vi "Panel.vi"(11 "ArrayHostPanel in":refnum<class "ArrayHostPanel.lvclass">) -> ()   [LabVIEW 2020, in "Nested.lvlib" / "ArrayHostPanel.lvclass"]
uses:
  ArrayHostPanel.lvclass
  OOPanel/Panel/Basic UI State.ctl
  OOPanel/Panel/Panel.lvclass
  OOPanel/OOPanel.lvlib
  OOPanel/ArrayManager/ArrayManager.lvclass
  ColorArrayPanel/ColorArrayPanel.lvclass
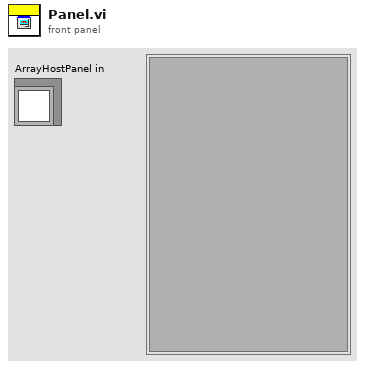
[diagram p1: front panel]
types:
  T1 = typedef "OOPanel.lvlib/Panel.lvclass/Basic UI State.ctl" = enum16{"Init", "Run", "Close"}
  T2 = typedef "OOPanel.lvlib/Panel.lvclass/Panel Events.ctl" = cluster{"Visbility":refnum<user-event>, "Close":refnum<user-event>}
  T3 = typedef "OOPanel.lvlib/Visibility State.ctl" = enum16{"Idle", "Closed", "Hidden", "Visible", "Subpanel", "Hidden Subpanel"}
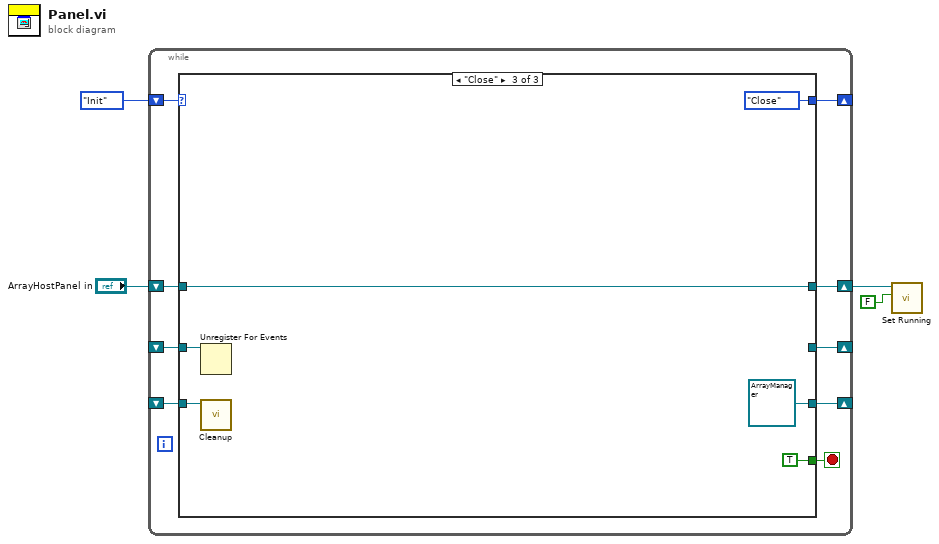
[diagram p0: block diagram]
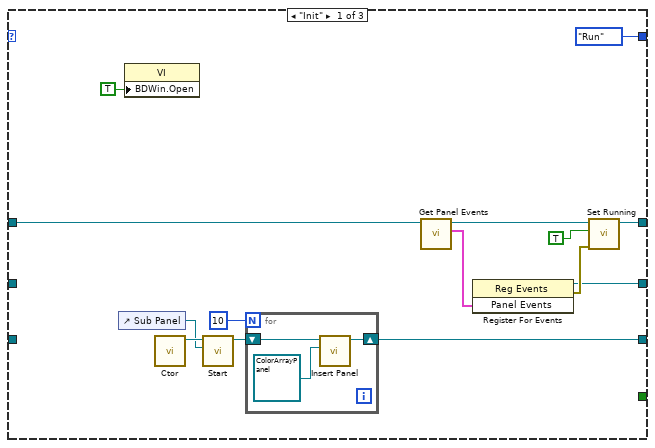
[diagram p2: hidden frame]
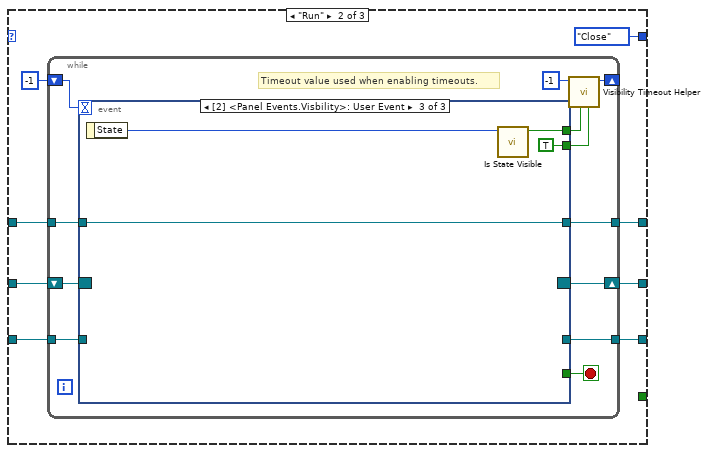
[diagram p3: hidden frame]
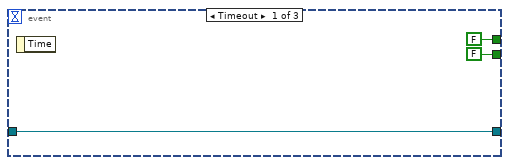
[diagram p4: hidden frame]
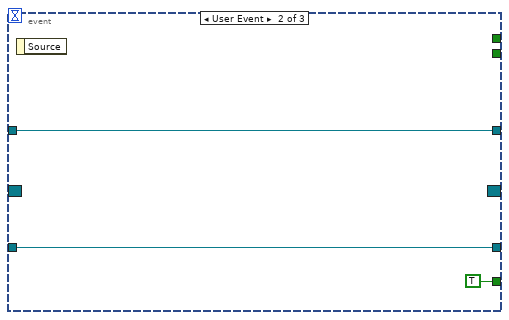
[diagram p5: hidden frame]
diagram:
  n1 = while {
    shift-right: [w12] -> _
    shift-left: _ -> [w13]
    shift-right: [w10] -> _
    shift-left: Basic_UI_State."Init" ("Basic UI State") -> [w11]
    shift-right: [w8] -> w1
    shift-left: "ArrayHostPanel in" -> [w7]
    shift-right: [w6] -> _
    shift-left: _ -> [w5]
    stop <- w9 stop-if-true
    n2 = case shown="\"Close\"" w11 {
      tunnel: w13 -> [_ w38 w64]
      tunnel: [w24 w36 _] -> w12
      tunnel: [Basic_UI_State."Run" ("Basic UI State") Basic_UI_State."Close" ("Basic UI State") Basic_UI_State."Close" ("Basic UI State")] -> w10
      tunnel: [_ _ TRUE] -> w9
      tunnel: [w23 w33 w61] -> w8
      tunnel: w7 -> [w22 w34 w61]
      tunnel: [w15 w31 refnum<class "ArrayManager.lvclass"> refnum ("ArrayManager out")] -> w6
      tunnel: w5 -> [_ w32 w63]
      frame "Init" {
        n3 = control-ref of="Sub Panel"() -> (w17:refnum<vi>)
        n4 = property class="VI"("BDWin.Open"=TRUE ("Block Diagram Window:Open")) -> ()  [unwired: 2 in, 2 out]
        n5 = call "Ctor.vi"() -> ("PanelArray"=w18:refnum<class "ArrayManager.lvclass">)  [unwired: 10 in, 1 out]
        n6 = call "Start.vi"("Container"=w17, "ArrayManager in"=w18) -> ("ArrayManager out"=w16:refnum<class "ArrayManager.lvclass">)  [unwired: 8 in, 1 out]
        n7 = for {
          N: 10 -> [_]
          shift-right: [w28] -> w15
          shift-left: w16 -> [w30]
          n8 = call "Insert Panel.vi"("Panel/Type"=refnum<class "ColorArrayPanel.lvclass"> refnum ("Nested.lvlib:ColorArrayPanel.lvclass"), "PanelArray in"=w30) -> ("PanelArray out"=w28:refnum<class "ArrayManager.lvclass">)  [unwired: 7 in, 2 out]
        }
        n9 = call "Get Panel Events.vi"("Panel in"=w22) -> ("Panel Events"=w20:T2, "Panel out"=w21:refnum<class "ArrayHostPanel.lvclass">)  [unwired: 8 in, 1 out]
        n10 = register-events(w20) -> (reference out=w24:refnum<event-registration>, error out=w26:errorcluster)  [unwired: 2 in]
        n11 = call "Set Running.vi"("error in (no error)"=w26, "Running"=TRUE, "Panel in"=w21) -> ("Panel out"=w23:refnum<class "ArrayHostPanel.lvclass">)  [unwired: 7 in, 1 out]
      }
      frame "Run" {
        n12 = while {
          shift-right: [w46] -> w36
          shift-left: w38 -> [w47]
          shift-right: [w49] -> _
          shift-left: -1 ("Timeout") -> [w48]
          tunnel: w34 -> [w42]
          tunnel: [w41] -> w33
          tunnel: w32 -> [w40]
          tunnel: [w39] -> w31
          stop <- w43 stop-if-true
          # "Timeout value used when enabling timeouts."
          n13 = event shown="[2] <Panel Events.Visbility>: User Event" {
            selector: w47 -> [_ _ _]
            dyn-events: [_ _ _] -> w46
            timeout: w48 -> [_ _ _]
            tunnel: [FALSE _ w59] -> w45
            tunnel: [FALSE _ TRUE] -> w44
            tunnel: [_ TRUE _] -> w43
            tunnel: w42 -> [w51 w55 w57]
            tunnel: [w51 w55 w57] -> w41
            tunnel: w40 -> [_ w54 _]
            tunnel: [_ w54 _] -> w39
            event Timeout {
              n14 = event-data() -> ()  [unwired: 1 in, 1 out]
            }
            event User Event {
              n15 = event-data() -> ()  [unwired: 1 in, 1 out]
            }
            event User Event {
              n16 = event-data() -> ("State"=w60:T3)  [unwired: 1 in]
              n17 = call "Is State Visible.vi"("Visibility"=w60) -> ("Visible"=w59:bool)  [unwired: 10 in]
            }
          }
          n18 = call "Visibility Timeout Helper.vi"("Update?"=w44, "Use Timeout?"=w45, "Visible Timeout mS"=-1) -> ("Timeout"=w49:i32)  [unwired: 8 in]
        }
      }
      frame "Close" {
        n19 = Unregister For Events(event registration refnum=w64) -> ()  [unwired: 1 in, 1 out]
        n20 = call "Cleanup.vi"("PanelArray in"=w63) -> ()  [unwired: 10 in, 1 out]
      }
    }
  }
  n21 = call "Set Running.vi"("Running"=FALSE, "Panel in"=w1) -> ()  [unwired: 8 in, 2 out]
